vi "Get client handle.vi"(8 "error in (no error)":errorcluster, 9 "headers":T1[](array[typedef]), 11 "REST Client in":refnum<class "REST Client.lvclass">) -> (0 "error out":errorcluster, 1 "headers out":T1[](array[typedef]), 2 "http-client":refnum<class "http-client.lvclass">, 3 "REST Client out":refnum<class "REST Client.lvclass">)   [LabVIEW 2020, in "REST Client.lvlib" / "REST Client.lvclass"]
uses:
  REST Client.lvclass
  http-client/http-client.lvclass
  HTTP Header.ctl
  <vilib>/NI/Advanced HTTP Client/Header--Combo Box.ctl
  REST Client.lvclass/REST Client.ctl
  <vilib>/NI/Advanced HTTP Client/Session.lvclass
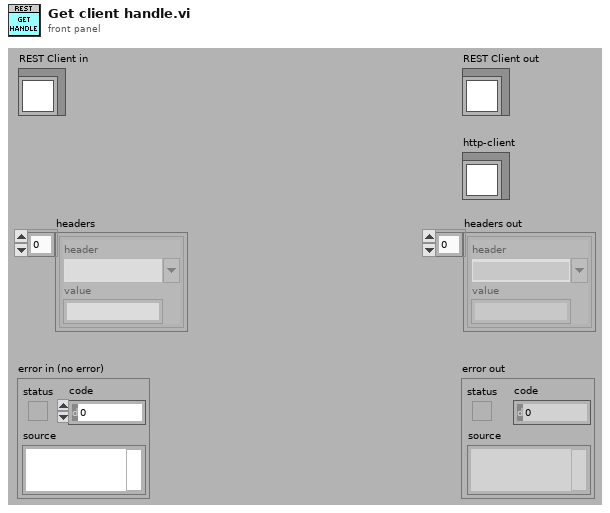
[diagram p1: front panel]
types:
  T1 = typedef "REST Client.lvlib/REST Client.lvclass/HTTP Header.ctl" = cluster{"header":T2, "value":string}
  T2 = typedef "lib_NI_Advanced HTTP Client.lvlib/Session.lvclass/Header--Combo Box.ctl" = string
  T3 = cluster{"session":refnum<class "http-client.lvclass">, "Default Headers ([JSON])":T1[]}
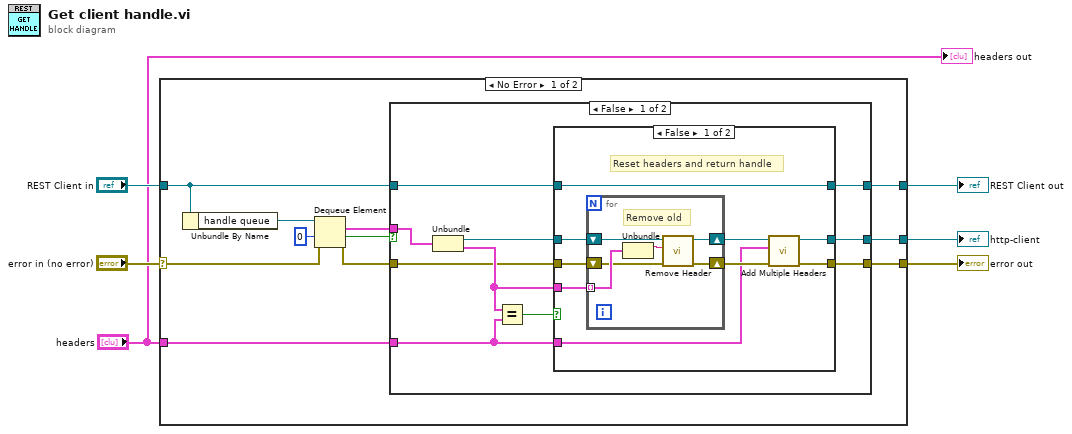
[diagram p0: block diagram]
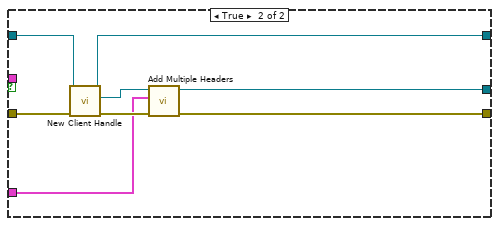
[diagram p3: hidden frame]
diagram:
  n1 = case shown="No Error" "error in (no error)" {
    selector: "error in (no error)" -> [w7 w54]
    tunnel: [w14 w54] -> w5
    tunnel: [w17 w55] -> w3
    tunnel: "REST Client in" -> [w13 w55]
    tunnel: [w15 _] -> w1
    tunnel: "headers" -> [w16 _]
    frame No Error {
      n2 = Unbundle By Name(w13) -> ("handle queue"=w12:refnum<queue>)
      n3 = Dequeue Element(queue=w12, timeout in ms (-1)=0, error in (no error)=w7) -> (element=w9:T3, timed out?=w10:bool, error out=w8:errorcluster)  [unwired: 1 out]
      n4 = case shown="False" w10 {
        tunnel: [w19 w51] -> w17
        tunnel: w16 -> [w24 w46]
        tunnel: [w23 w47] -> w15
        tunnel: [w22 w48] -> w14
        tunnel: w13 -> [w20 w52]
        tunnel: w8 -> [w21 w53]
        tunnel: w9 -> [w18 _]
        frame False {
          n5 = Unbundle(w18) -> ("session"=w26:refnum<class "http-client.lvclass">, "Default Headers ([JSON])"=w25:T1[])
          n6 = Equal?(x=w25, y=w24) -> (x = y?=w27:bool)
          n7 = case shown="False" w27 {
            tunnel: w26 -> [w34 w45]
            tunnel: w25 -> [w33 _]
            tunnel: w24 -> [w28 _]
            tunnel: [w31 w45] -> w23
            tunnel: [w30 w44] -> w22
            tunnel: w21 -> [w36 w44]
            tunnel: w20 -> [w35 w43]
            tunnel: [w35 w43] -> w19
            frame False {
              # "Reset headers and return handle"
              n8 = for {
                shift-right: [w37] -> w29
                shift-left: w36 -> [w39]
                shift-right: [w38] -> w32
                shift-left: w34 -> [w41]
                tunnel: w33 -> [w42] mode=indexing
                # "Remove old"
                n9 = Unbundle(w42) -> ("header"=w40:T2)  [unwired: 1 out]
                n10 = call "Remove Header.vi"("error in"=w39, "header"=w40, "http-client in"=w41) -> ("error out"=w37:errorcluster, "http-client out"=w38:refnum<class "http-client.lvclass">)  [unwired: 7 in]
              }
              n11 = call "Add Multiple Headers.vi"("error in"=w29, "headers"=w28, "http-client in"=w32) -> ("error out"=w30:errorcluster, "http-client out"=w31:refnum<class "http-client.lvclass">)  [unwired: 7 in]
            }
            frame True {
              # "Use existing handle"
            }
          }
        }
        frame True {
          n12 = call "New Client Handle.vi"("error in (no error)"=w53, "REST Client in"=w52) -> ("error out"=w49:errorcluster, "http-client"=w50:refnum<class "http-client.lvclass">, "REST Client out"=w51:refnum<class "REST Client.lvclass">)  [unwired: 7 in]
          n13 = call "Add Multiple Headers.vi"("error in"=w49, "headers"=w46, "http-client in"=w50) -> ("error out"=w48:errorcluster, "http-client out"=w47:refnum<class "http-client.lvclass">)  [unwired: 7 in]
        }
      }
    }
    frame Error {
    }
  }
  "error out" <- w5
  "REST Client out" <- w3
  "http-client" <- w1
  "headers out" <- "headers"
